vi "from string 1.0.vi"(8 "error in (no error)":errorcluster, 10 "data":string, 11 "E2E configuration in":refnum<class "E2E Tag Exchange configuration.lvclass">) -> (0 "error out":errorcluster, 3 "E2E configuration out":refnum<class "E2E Tag Exchange configuration.lvclass">)   [LabVIEW 2015, in "E2E Tag Exchange configuration.lvclass"]
uses:
  E2E Tag Exchange configuration.lvclass
  Runtime Implementation.ctl
  <vilib>/NI/Tag Bus Module Framework/channel/TBM channel.lvclass
  E2E Tag Exchange configuration.lvclass/E2E Tag Exchange configuration.ctl
  <vilib>/NI/Configuration Framework/serializable configuration/NISE_CEF_serializable configuration.lvclass
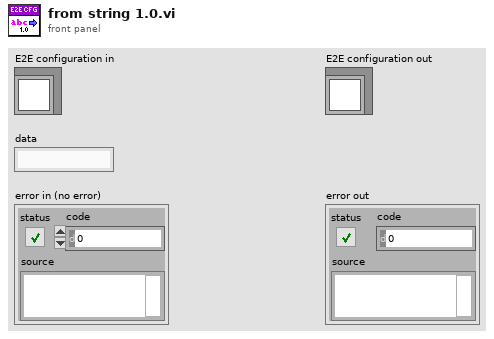
[diagram p1: front panel]
types:
  T1 = typedef "E2E Tag Exchange configuration.lvclass/Runtime Implementation.ctl" = enum16{"RT FIFO", "UDP"}
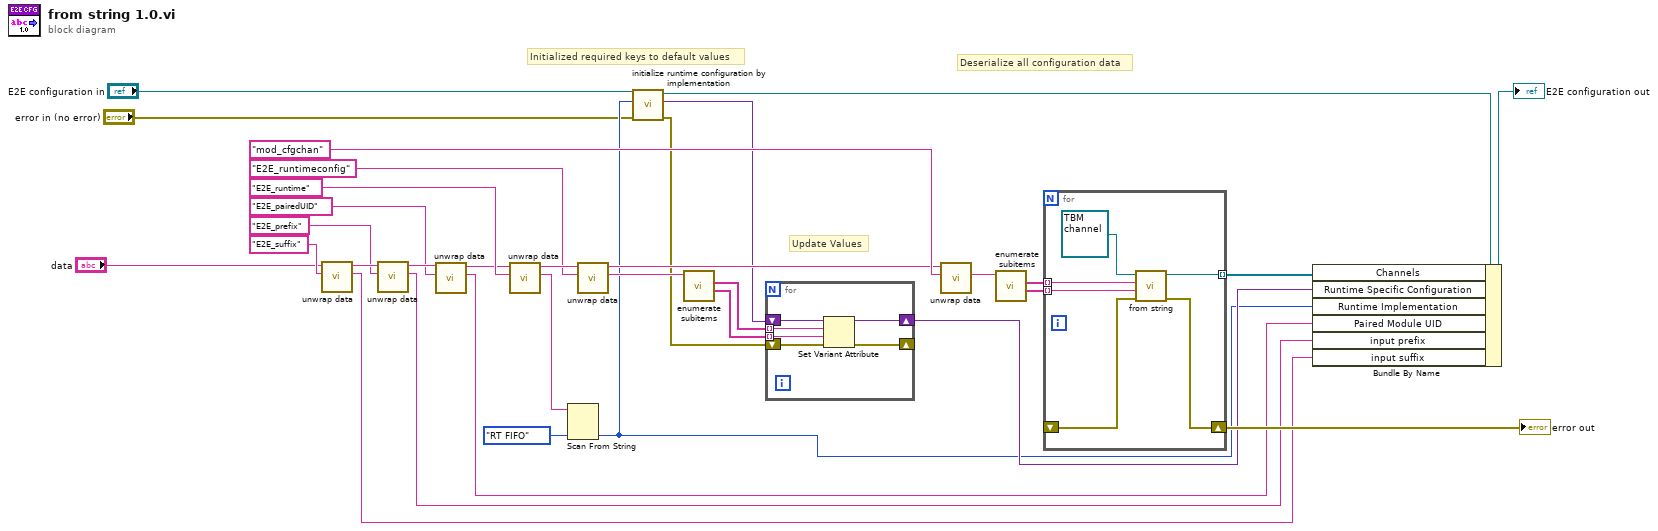
[diagram p0: block diagram]
diagram:
  # "Update Values"
  # "Initialized required keys to default values"
  # "Deserialize all configuration data"
  n1 = call <vilib>:"unwrap data.vi"("identifier"="E2E_suffix", "data to unwrap"="data") -> ("unwrapped data"=w18:string, "remaining string"=w20:string)  [unwired: 8 in]
  n2 = call <vilib>:"unwrap data.vi"("identifier"="E2E_prefix", "data to unwrap"=w20) -> ("unwrapped data"=w21:string, "remaining string"=w19:string)  [unwired: 8 in]
  n3 = call <vilib>:"unwrap data.vi"("identifier"="E2E_pairedUID", "data to unwrap"=w19) -> ("unwrapped data"=w22:string, "remaining string"=w23:string)  [unwired: 8 in]
  n4 = call <vilib>:"unwrap data.vi"("identifier"="E2E_runtime", "data to unwrap"=w23) -> ("unwrapped data"=w25:string, "remaining string"=w11:string)  [unwired: 8 in]
  n5 = Scan From String(input string=w25, default 1=Runtime_Implementation."RT FIFO" ("Runtime Implementation")) -> (output 1=w6:T1)  [unwired: 3 in, 3 out]
  n6 = call <vilib>:"unwrap data.vi"("identifier"="E2E_runtimeconfig", "data to unwrap"=w11) -> ("unwrapped data"=w9:string, "remaining string"=w10:string)  [unwired: 8 in]
  n7 = call "initialize runtime configuration by implementation.vi"("error in (no error)"="error in (no error)", "Runtime Implementation"=w6, "E2E configuration in"="E2E configuration in") -> ("error out"=w1:errorcluster, "Runtime Specific Configuration"=w2:variant, "E2E configuration out"=w3:refnum<class "E2E Tag Exchange configuration.lvclass">)  [unwired: 6 in]
  n8 = call <vilib>:"enumerate subitems.vi"("data to enumerate"=w9) -> ("associated data"=w12:string[], "discovered subitems"=w13:string[])  [unwired: 8 in, 1 out]
  n9 = for {
    shift-right: [w36] -> w7
    shift-left: w2 -> [w39]
    tunnel: w13 -> [w38] mode=indexing
    tunnel: w12 -> [w37] mode=indexing
    shift-right: [w34] -> _
    shift-left: w1 -> [w35]
    n10 = Set Variant Attribute(Variant=w39, name=w38, value=w37, error in=w35) -> (Variant out=w36:variant, error out=w34:errorcluster)  [unwired: 1 out]
  }
  n11 = call <vilib>:"unwrap data.vi"("identifier"="mod_cfgchan", "data to unwrap"=w10) -> ("unwrapped data"=w32:string)  [unwired: 8 in, 1 out]
  n12 = call <vilib>:"enumerate subitems.vi"("data to enumerate"=w32) -> ("associated data"=w31:string[], "discovered subitems"=w30:string[])  [unwired: 8 in, 1 out]
  n13 = for {
    shift-right: [w45] -> w33
    shift-left: _ -> [w44]
    tunnel: w30 -> [w43] mode=indexing
    tunnel: w31 -> [w42] mode=indexing
    tunnel: [w40] -> w27 mode=indexing
    n14 = call-dynamic "from string.vi"("error in"=w44, "channel data"=w42, "identifier"=w43, "channel in"=refnum<class "TBM channel.lvclass"> refnum) -> ("error out"=w45:errorcluster, "channel out"=w40:refnum<class "TBM channel.lvclass">)  [unwired: 6 in]
  }
  "error out" <- w33
  n15 = Bundle By Name(cluster=w3, "Channels"=w27, "Runtime Specific Configuration"=w7, "Runtime Implementation"=w6, "Paired Module UID"=w22, "input prefix"=w21, "input suffix"=w18) -> (→"E2E configuration out":refnum<class "E2E Tag Exchange configuration.lvclass">)
